vi "Variant_SetName.vi"(10 "Name":string, 11 "Variant":variant) -> (3 "Named Variant":variant)   [LabVIEW 2013, in "OpenVariant.lvlib"]
uses:
  OpenVariant.lvlib
  <vilib>/Utility/VariantDataType/TypedefInfo.ctl
  TypeDescriptor/OpenDescriptor.lvlib
  <vilib>/Utility/VariantDataType/VariantType.lvlib
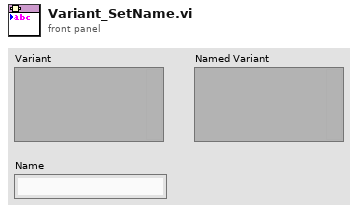
[diagram p1: front panel]
types:
  T1 = typedef "VariantType.lvlib/TypedefInfo.ctl" = cluster{"Name":string, "Timestamp":u32}
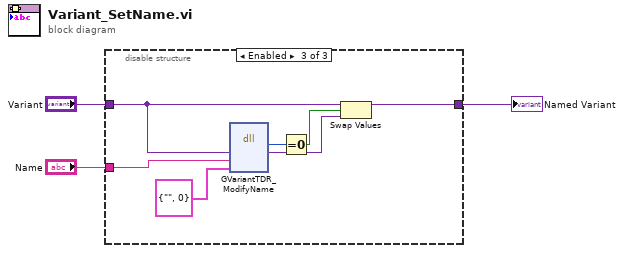
[diagram p0: block diagram]
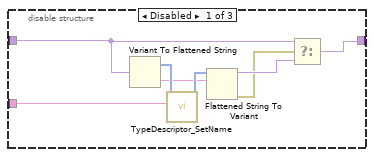
[diagram p2: hidden frame]
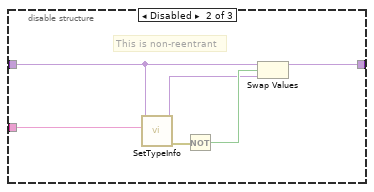
[diagram p3: hidden frame]
diagram:
  n1 = disable-structure shown="Enabled" {
    disable-tunnel: "Name" -> [w9 w17 w24]
    disable-tunnel: "Variant" -> [w7 w13 w22]
    disable-tunnel: [w5 w14 w20] -> w1
    frame Disabled {
      n2 = Variant To Flattened String(Variant=w7) -> (data string=w8:string, 1:w10:i16[])
      n3 = call "TypeDescriptor_SetName.vi"("name"=w9, "type descriptor"=w10) -> ("type descriptor dup"=w11:i16[])  [unwired: 7 in, 2 out]
      n4 = Flattened String To Variant(6:w8, 7:w11) -> (0:w4:errorcluster, 3:w6:variant)  [unwired: 1 in]
      n5 = Select(t=w7, s=w4, f=w6) -> (s? t:f=w5:variant)
    }
    frame Disabled {
      # "This is non-reentrant"
      n6 = call <vilib>:"SetTypeInfo.vi"("Name"=w17, "Variant"=w13) -> ("error out"=w16:errorcluster, "Variant Out"=w12:variant)  [unwired: 8 in]
      n7 = Not(x=w16) -> (.not. x?=w15:bool)
      n8 = Swap Values(12:w13, 13:w15, 14:w12) -> (1:w14:variant)  [unwired: 1 out]
    }
    frame Enabled {
      n9 = dll-call lib="LabVIEW" fn="GVariantTDR_ModifyName"("lvVarInOut"=w22, "nameIn"=w24, "typeDefIn"=T1 {"Name"="", "Timestamp"=0}) -> ("return type"=w19:i32, "lvVarInOut"=w21:variant)  [unwired: 5 in, 2 out]
      n10 = Equal To 0?(x=w19) -> (x = 0?=w18:bool)
      n11 = Swap Values(12:w22, 13:w18, 14:w21) -> (1:w20:variant)  [unwired: 1 out]
    }
  }
  "Named Variant" <- w1
